vi "Add Bouton.vi"(8 "error in (no error)":errorcluster, 9 "Arguments":string, 10 "Content":string, 11 "ToastBuilder in":refnum<class "ToastBuilder.lvclass">) -> (0 "error out":errorcluster, 3 "ToastBuilder out":refnum<class "ToastBuilder.lvclass">)   [LabVIEW 2026, in "ToastNotification.lvlib" / "ToastBuilder.lvclass"]
doc: "Add a button to the native builder. Content is the visible button label; Arguments is the raw activation string returned when the button is clicked, for example action=Reply. Call before Show. The operation is skipped on incoming error and preserves the input builder. This overload does not expose a text-input association or activation-type option. Native object lifetime hardening remains part of the documented follow-up work."
uses:
  ToastBuilder.lvclass
  ToastBuilder.lvclass/ToastBuilder.ctl
  Read Builder Reference.vi
  Write Builder Reference.vi
  Toast Native/Toast Native.lvlib
  Reflection DotNet/Reflection DotNet.lvlib
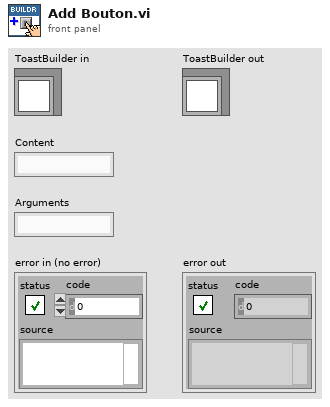
[diagram p1: front panel]
types:
  T1 = typedef "ToastNotification.lvlib/ToastBuilder.lvclass/Builder Reference.ctl" = refnum<k24>
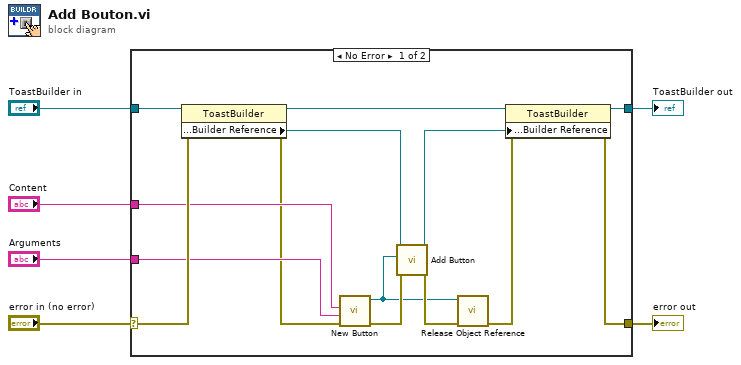
[diagram p0: block diagram]
diagram:
  n1 = case shown="No Error" "error in (no error)" {
    selector: "error in (no error)" -> [w17 w22]
    tunnel: [w16 w22] -> w5
    tunnel: [w18 w21] -> w3
    tunnel: "ToastBuilder in" -> [w20 w21]
    tunnel: "Arguments" -> [w11 _]
    tunnel: "Content" -> [w12 _]
    frame No Error {
      n2 = property class="ToastBuilder"(reference=w20, error in=w17) -> (reference out=w19:refnum<class "ToastBuilder.lvclass">, error out=w10:errorcluster, "Public:Properties:Builder Reference"=w14:T1)
      n3 = call "New Button.vi"("error in (no error)"=w10, "arguments"=w11, "content"=w12) -> ("error out"=w15:errorcluster, "new reference"=w7:refnum<k24>)  [unwired: 7 in]
      n4 = call "Add Button.vi"("error in (no error)"=w15, "button"=w7, "reference"=w14) -> ("error out"=w9:errorcluster, "reference out"=w13:refnum<k24>)  [unwired: 7 in]
      n5 = call "Release Object Reference.vi"("error in"=w9, "object"=w7) -> ("error out"=w8:errorcluster)  [unwired: 9 in]
      n6 = property class="ToastBuilder"(reference=w19, error in=w8, "Public:Properties:Builder Reference"=w13) -> (reference out=w18:refnum<class "ToastBuilder.lvclass">, error out=w16:errorcluster)
    }
    frame Error {
    }
  }
  "error out" <- w5
  "ToastBuilder out" <- w3
